vi "Add Resolver.vi"(8 "error in (no error)":errorcluster, 9 "Namespace":string, 10 "Resolver":refnum<class "TemplateValueResolver.lvclass">, 11 "BasicTemplater in":refnum<class "BasicTemplater.lvclass">) -> (0 "error out":errorcluster, 3 "BasicTemplater out":refnum<class "BasicTemplater.lvclass">)   [LabVIEW 2020, in "HTTP Server.lvlib" / "BasicTemplater.lvclass"]
uses:
  BasicTemplater.lvclass
  TemplateVariableResolver/TemplateValueResolver.lvclass
  BasicTemplater.lvclass/BasicTemplater.ctl
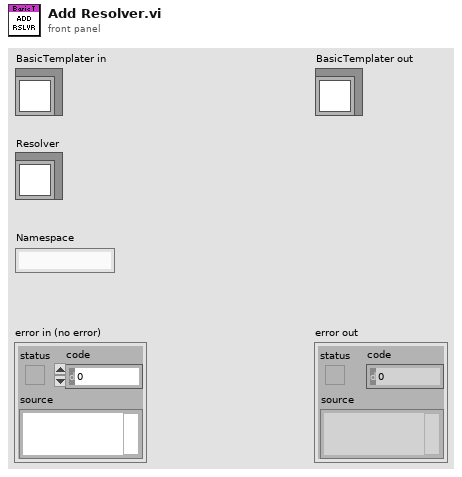
[diagram p1: front panel]
types:
  T1 = map{string, refnum<class "TemplateValueResolver.lvclass">}
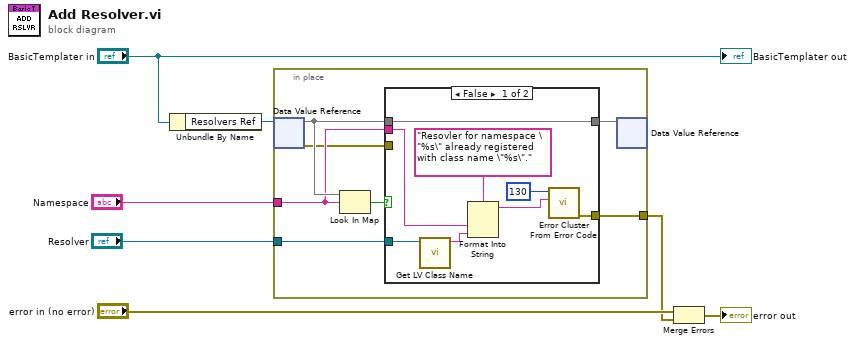
[diagram p0: block diagram]
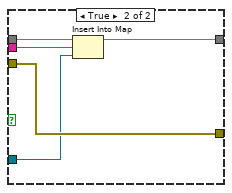
[diagram p2: hidden frame]
diagram:
  n1 = Unbundle By Name("BasicTemplater in") -> ("Resolvers Ref"=w6:refnum<data-value>)
  n2 = in-place {
    in-place-border: "Namespace" -> [w12]
    in-place-border: "Resolver" -> [w11]
    in-place-border: [w9] -> w1
    n3 = in-place-dvr #1(w6) -> (w13:T1, w8:errorcluster)
    n4 = Look In Map(map=w13, key=w12) -> (key not found?=w14:bool)  [unwired: 1 in, 1 out]
    n5 = case shown="False" w14 {
      tunnel: w13 -> [w22 w26]
      tunnel: w12 -> [w20 w25]
      tunnel: w11 -> [w18 w24]
      tunnel: [w22 w23] -> w10
      tunnel: [w15 w27] -> w9
      tunnel: w8 -> [_ w27]
      frame False {
        n6 = call <vilib>:"Get LV Class Name.vi"("object"=w18) -> ("class name"=w17:string)  [unwired: 9 in, 1 out]
        n7 = Format Into String(format string="Resovler for namespace \"%s\" already registered with class name \"%s\".", w20, w17) -> (resulting string=w16:string)  [unwired: 2 in, 1 out]
        n8 = call <vilib>:"Error Cluster From Error Code.vi"("error message (\"\")"=w16, "error code (0)"=130) -> ("error out"=w15:errorcluster)  [unwired: 7 in]
      }
      frame True {
        n9 = Insert Into Map(map in=w26, key=w25, value=w24) -> (map out=w23:T1)  [unwired: 2 out]
      }
    }
    n10 = in-place-dvr #1(w10) -> ()  [unwired: 2 out]
  }
  n11 = Merge Errors("error in (no error)", w1) -> (→"error out":errorcluster)
  "BasicTemplater out" <- "BasicTemplater in"
